vi "Corporate Actions.vi"(11 "market":T1) -> (3 "market out":T1)   [LabVIEW 2020, in "Full Featured MCP Server.lvlib"]
doc: "Keeps prices in a sensible range however long the server runs. A stock that has risen to 10 times its start price is split 5 for 1: the price and its history are divided by five and every owned share becomes five. A stock that has fallen to a 10th of its start price goes insolvent: owned shares are lost and a successor is listed at 10 times the price. Both are published as news; the history is rescaled so charts and percent changes stay continuous."
uses:
  Full Featured MCP Server.lvlib
  Market State.ctl
  News Item.ctl
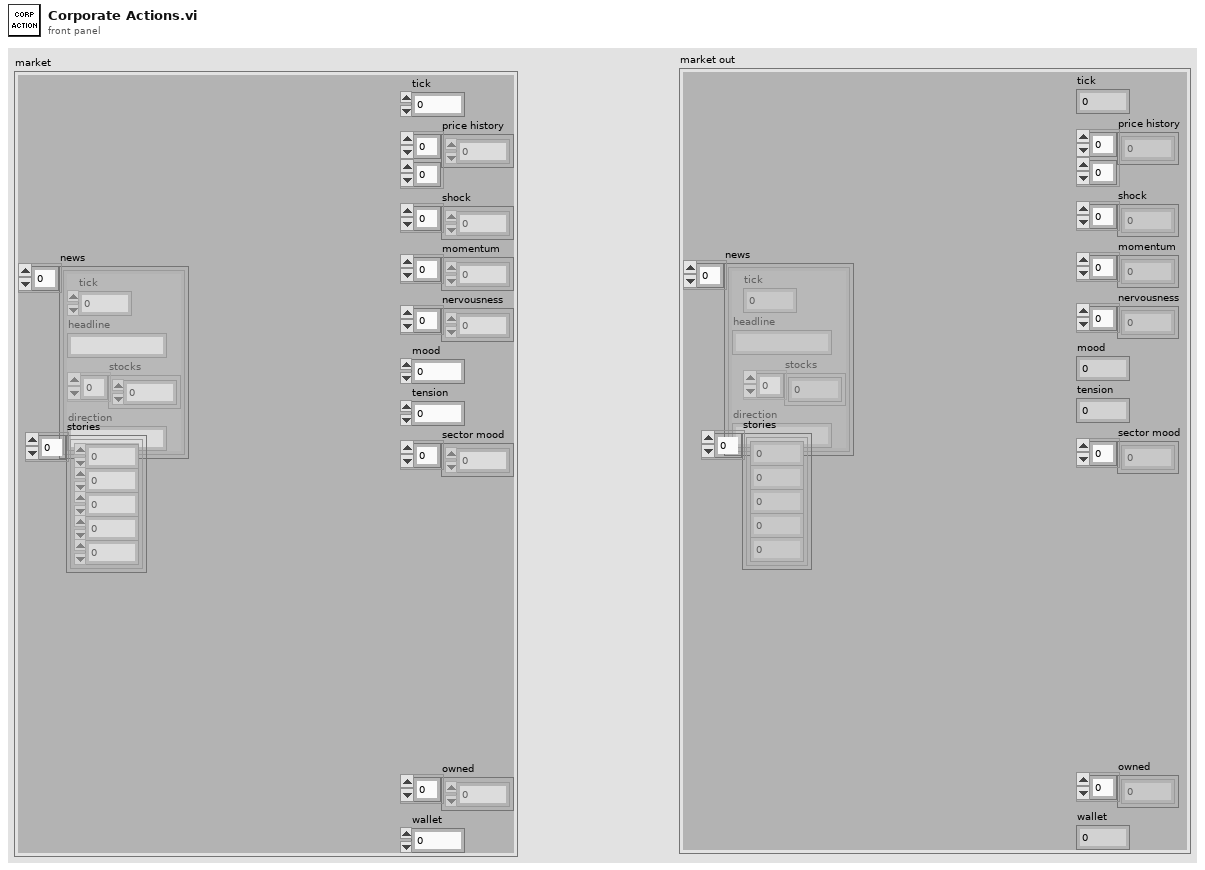
[diagram p1: front panel]
types:
  T1 = typedef "Full Featured MCP Server.lvlib/Market State.ctl" = cluster{"tick":i32, "price history":dbl[][], "shock":dbl[], "momentum":dbl[], "nervousness":dbl[], "mood":dbl, "tension":dbl, "sector mood":dbl[], "news":T2[], "stories":cluster{"arc":i32, "step":i32, "due":i32, "stock":i32, "other":i32}[], "owned":i32[], "wallet":dbl}
  T2 = typedef "Full Featured MCP Server.lvlib/News Item.ctl" = cluster{"tick":i32, "headline":string, "stocks":i32[], "direction":string}
  T3 = cluster{"name":string, "sector":i32, "quality":i32, "start price":dbl, "drift":dbl, "volatility":dbl, "beta":dbl, "jumpiness":dbl, "description":string}[]
  T4 = cluster{"headline":string, "scope":enum16{"one stock", "two stocks", "sector", "market"}, "direction":string, "jump":dbl, "follow":dbl, "jump other":dbl, "follow other":dbl}[]
  T5 = cluster{"headline":string, "scope":enum16{"one stock", "two stocks", "sector", "market"}, "direction":string, "jump":dbl, "follow":dbl, "jump other":dbl, "follow other":dbl}
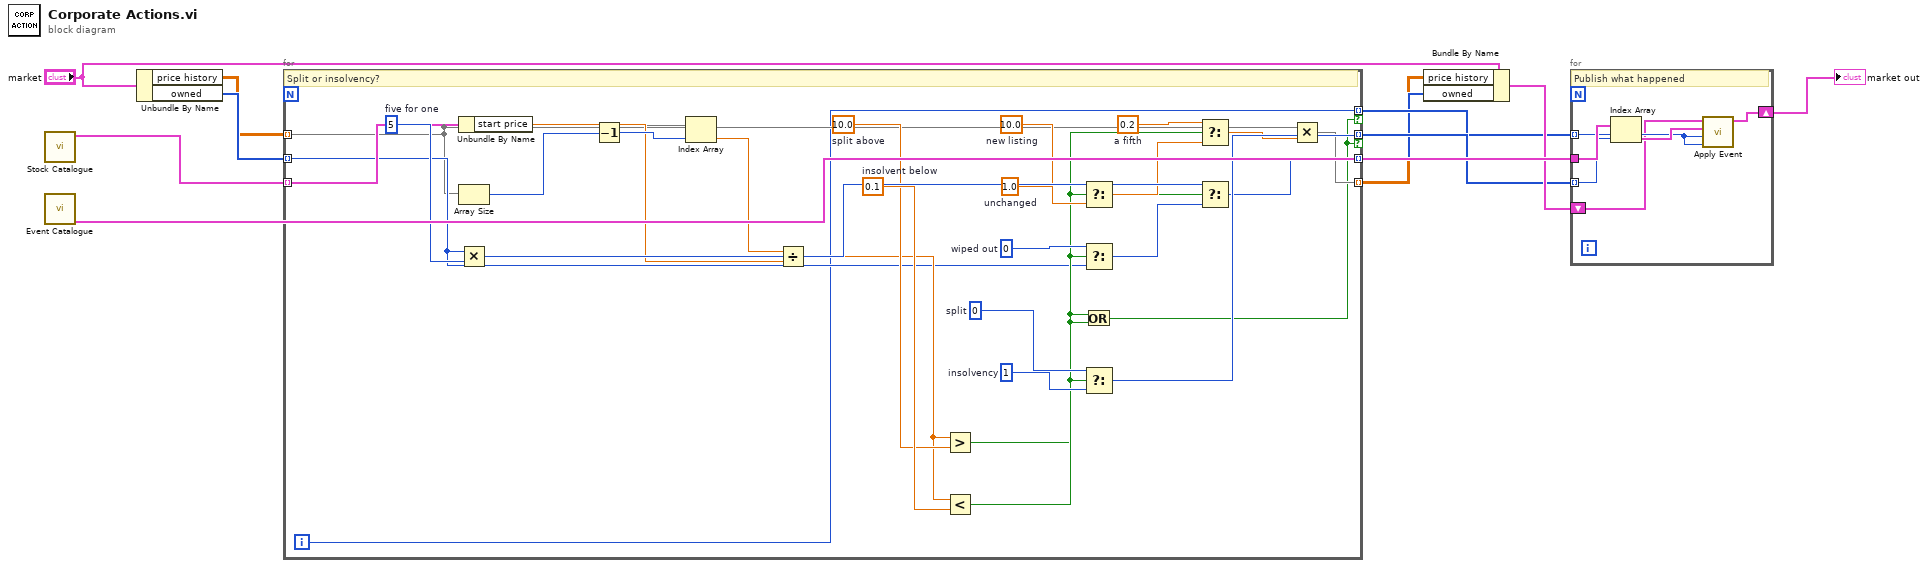
[diagram p0: block diagram]
diagram:
  n1 = call "Stock Catalogue.vi"() -> ("stocks"=w4:T3)  [unwired: 10 in, 1 out]
  n2 = call "Event Catalogue.vi"() -> ("corporate actions"=w10:T4)  [unwired: 8 in, 3 out]
  n3 = Unbundle By Name("market") -> ("price history"=w2:dbl[][], "owned"=w3:i32[])
  n4 = for {
    tunnel: [w12] -> w7 mode=indexing if=w35
    tunnel: w2 -> [w13] mode=indexing
    tunnel: w3 -> [w14] mode=indexing
    tunnel: w4 -> [w15] mode=indexing
    tunnel: [w39] -> w8 mode=indexing if=w35
    tunnel: [w34] -> w6 mode=indexing
    tunnel: [w36] -> w5 mode=indexing
    i -> [w12]
    w38 = 1  # insolvency
    w37 = 0  # split
    w32 = 0  # wiped out
    w30 = 5  # five for one
    w27 = 1.0  # unchanged
    w26 = 10.0  # new listing
    w25 = 0.2  # a fifth
    w23 = 0.1  # insolvent below
    w21 = 10.0  # split above
    # "Split or insolvency?"
    n5 = Unbundle By Name(w15) -> ("start price"=w16:dbl)
    n6 = Array Size(array=w13) -> (size(s)=w17:i32)
    n7 = Multiply(x=w14, y=w30) -> (x*y=w31:i32)
    n8 = Decrement(x=w17) -> (x-1=w18:i32)
    n9 = Index Array(array=w13, index=w18) -> (element=w19:dbl)
    n10 = Divide(x=w19, y=w16) -> (x/y=w20:dbl)
    n11 = Greater?(x=w20, y=w21) -> (0:w22:bool)
    n12 = Less?(x=w20, y=w23) -> (x < y?=w24:bool)
    n13 = Select(t=w26, s=w24, f=w27) -> (s? t:f=w28:dbl)
    n14 = Select(t=w32, s=w24, f=w14) -> (s? t:f=w33:i32)
    n15 = Or(x=w22, y=w24) -> (x .or. y?=w35:bool)
    n16 = Select(t=w37, s=w22, f=w38) -> (s? t:f=w39:i32)
    n17 = Select(t=w25, s=w22, f=w28) -> (s? t:f=w29:dbl)
    n18 = Select(t=w31, s=w22, f=w33) -> (s? t:f=w34:i32)
    n19 = Multiply(x=w13, y=w29) -> (x*y=w36:dbl[])
  }
  n20 = Bundle By Name(cluster="market", "price history"=w5, "owned"=w6) -> (w9:T1)
  n21 = for {
    tunnel: w7 -> [w42] mode=indexing
    tunnel: w10 -> [w44]
    tunnel: w8 -> [w43] mode=indexing
    shift-right: [w41] -> w11
    shift-left: w9 -> [w40]
    # "Publish what happened"
    n22 = Index Array(array=w44, index=w43) -> (element=w45:T5)
    n23 = call "Apply Event.vi"("other"=w42, "stock"=w42, "event"=w45, "market"=w40) -> ("market out"=w41:T1)  [unwired: 7 in]
  }
  "market out" <- w11
